vi "Example SPI ADXL345.vi"() -> ()   [LabVIEW 2021]
uses:
  <vilib>/platform/TimedLoop/XDataNode/XDataNode.xnode
  <vilib>/Platform/TimedLoop/XDataNode/nitl_modes.ctl
  <vilib>/Platform/TimedLoop/XDataNode/XDNodeRunTimeDep.lvlib
  <vilib>/Platform/TimedLoop/XDataNode/wakeup.ctl
  <vilib>/Platform/TimedLoop/XDataNode/timing_clust.ctl
  wiringPi.lvlib
  Type Defs/SPI Dev.ctl
  Type Defs/SPI Channel.ctl
  Type Defs/SPI Device.ctl
panel:
  in  "SPI Device":T1
  out "Aceleration":cluster{dbl, dbl, dbl}(graph)
  in  "stop":bool
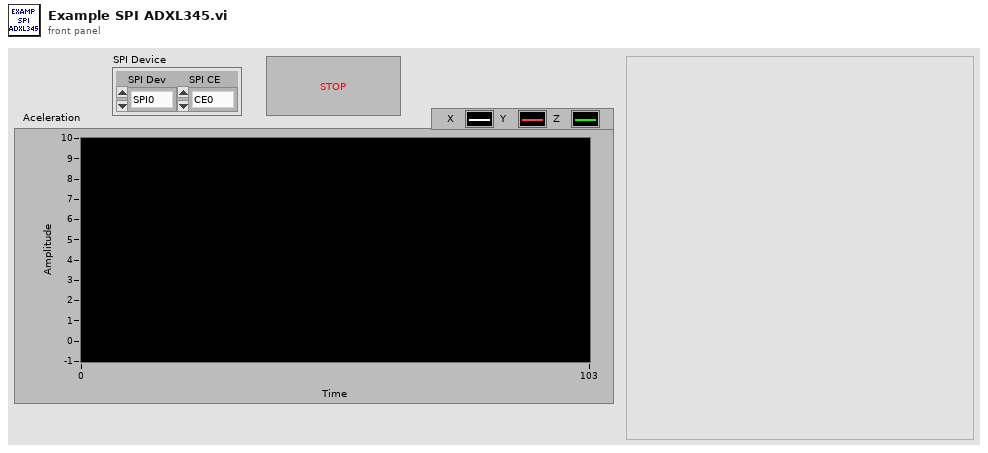
[diagram p1: front panel]
types:
  T1 = typedef "wiringPi.lvlib/SPI Device.ctl" = cluster{"SPI Dev":T2, "SPI CE":T3}
  T2 = typedef "wiringPi.lvlib/SPI Dev.ctl" = enum32{"SPI0", "SPI1"}
  T3 = typedef "wiringPi.lvlib/SPI Channel.ctl" = enum32{"CE0", "CE1", "CE2"}
  T4 = enum8{"DEVID", "-1-", "-2-", "-3-", "-4-", "-5-", "-6-", "-7-", "-8-", "-9-", "-A-", "-B-", "-C-", "-D-", "-E-", "-F-", "-10-", "-11-", "-12-", "-13-", "-14-", "-15-", "-16", "-17", "-18-", "-19-", "-1A-", "-1B-", "-1C-", "THRESH_TAP", "OFSX", "OFSY", "OFSZ", "DUR", "Latent", "Window", "THRESH_ACT", "THRESH_INACT", "TIME_INACT", "ACT_INACT_CTL", "THRESH_FF", "TIME_FF", "TAP_AXES", "ACT_TAP_STATUS", "BW_RATE", "POWER_CTL", "INT_ENABLE", "INT_MAP", "INT_SOURCE", "DATA_FORMAT", "DATAX0", "DATAX1", "DATAY0", "DATAY1", "DATAZ0", "DATAZ1", "FIFO_CTL", "FIFO_STATUS"}
  T5 = typedef "XDNodeRunTimeDep.lvlib/timing_clust.ctl" = cluster{"Expected End [f-1]":u64, "Actual End [f-1]":u64, "Finished Late? [f-1]":bool, "Expected End [i-1]":u64, "Actual End [i-1]":u64, "Finished Late? [i-1]":bool, "Expected Start [i]":u64, "Actual Start [i]":u64, "Expected Start [f]":u64, "Actual Start [f]":u64, "Source Name":string, "Structure Name":string, "Period":i64, "Deadline":i64, "Offset":i64, "Start":i64, "Priority":i32, "Timeout":i32, "Mode":T6, "Wakeup Reason":T7, "Error":errorcluster, "Source Type":string, "Secondary Source Type":string, "Global End Time":u64, "Global Start Time":u64, "Frame Duration":u64, "Iteration Duration":u64, "Assigned CPU":i32, "I/O Scan Engine Mode":u32}
  T6 = typedef "XDNodeRunTimeDep.lvlib/nitl_modes.ctl" = enum32{"No Change", "Process missed periods, maintain original phase", "Discard missed periods, maintain original phase", "Process missed periods, ignore original phase", "Discard missed periods, ignore original phase"}
  T7 = typedef "XDNodeRunTimeDep.lvlib/wakeup.ctl" = enum32{"Normal", "Aborted", "Asynchronous wakeup", "Timing source error", "Timed loop error", "Timeout"}
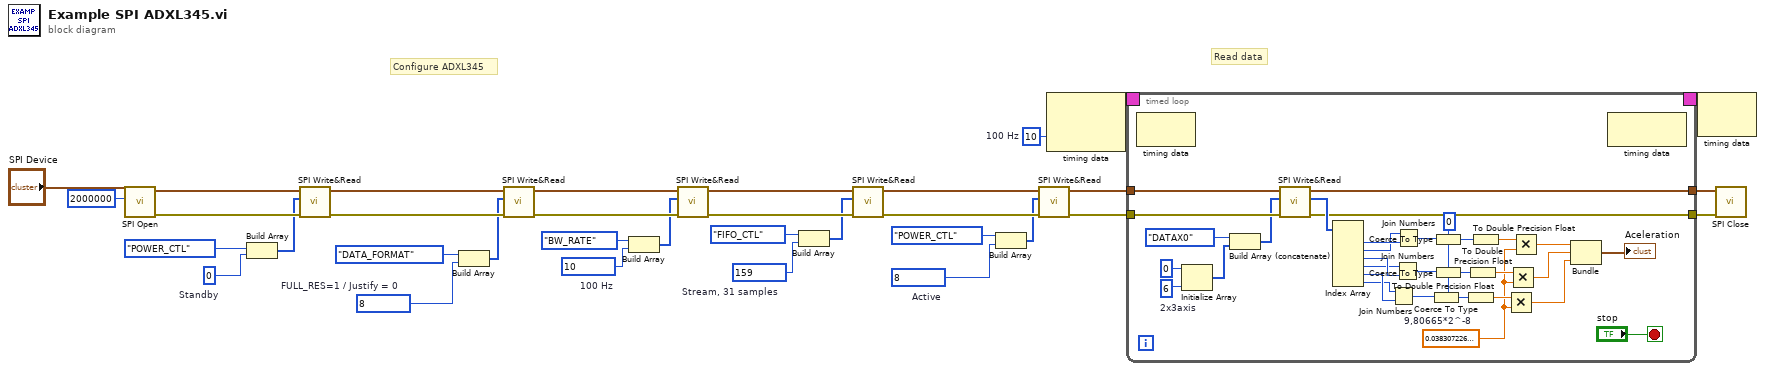
[diagram p0: block diagram]
diagram:
  w26 = i64 10  # 100 Hz
  w13 = u8 10  # 100 Hz
  w8 = u8 159  # Stream, 31 samples
  w17 = u8 8  # FULL_RES=1 / Justify = 0
  w6 = u8 8  # Active
  w21 = u8 0  # Standby
  # "Read data"
  # "Configure ADXL345"
  n1 = call "SPI Open.vi"("Speed"=2000000, "SPI Device"="SPI Device") -> ("error out"=w34:errorcluster, "SPI Device out"=w19:T1)  [unwired: 8 in]
  n2 = Build Array(T4."POWER_CTL" ("Dirección"), w21) -> (w20:u8[])
  n3 = call "SPI Write&Read.vi"("error in (no error)"=w34, "Data to Write"=w20, "SPI Device"=w19) -> ("error out"=w29:errorcluster, "SPI Device out"=w15:T1)  [unwired: 6 in, 1 out]
  n4 = Build Array(T4."DATA_FORMAT" ("Dirección"), w17) -> (w16:u8[])
  n5 = call "SPI Write&Read.vi"("error in (no error)"=w29, "Data to Write"=w16, "SPI Device"=w15) -> ("error out"=w33:errorcluster, "SPI Device out"=w14:T1)  [unwired: 6 in, 1 out]
  n6 = Build Array(T4."BW_RATE" ("Dirección"), w13) -> (w11:u8[])
  n7 = call "SPI Write&Read.vi"("error in (no error)"=w33, "Data to Write"=w11, "SPI Device"=w14) -> ("error out"=w31:errorcluster, "SPI Device out"=w3:T1)  [unwired: 6 in, 1 out]
  n8 = Build Array(T4."FIFO_CTL" ("Dirección"), w8) -> (w10:u8[])
  n9 = call "SPI Write&Read.vi"("error in (no error)"=w31, "Data to Write"=w10, "SPI Device"=w3) -> ("error out"=w32:errorcluster, "SPI Device out"=w4:T1)  [unwired: 6 in, 1 out]
  n10 = Build Array(T4."POWER_CTL" ("Dirección"), w6) -> (w5:u8[])
  n11 = call "SPI Write&Read.vi"("error in (no error)"=w32, "Data to Write"=w5, "SPI Device"=w4) -> ("error out"=w30:errorcluster, "SPI Device out"=w2:T1)  [unwired: 6 in, 1 out]
  n12 = node-c288(w26) -> (w28:T5)  [unwired: 1 in]
  n13 = timed-loop {
    timing: w28 -> [_]
    timing-out: [_] -> w27
    tunnel: w30 -> [w66]
    tunnel: [w46] -> w1
    tunnel: [w45] -> w25
    tunnel: w2 -> [w40]
    stop <- "stop" stop-if-true
    w51 = i16 0 ("number")
    w48 = 0.0383072265625  # 9,80665*2^-8
    w38 = u32 6  # 2x3axis
    n14 = node-c288() -> ()  [unwired: 1 in, 1 out]
    n15 = Initialize Array(u8 0 ("element"), w38) -> (w36:u8[])
    n16 = Build Array (concatenate)(T4."DATAX0" ("Address"), w36) -> (w35:u8[])
    n17 = call "SPI Write&Read.vi"("error in (no error)"=w66, "Data to Write"=w35, "SPI Device"=w40) -> ("error out"=w45:errorcluster, "Data readed"=w62:u8[], "SPI Device out"=w46:T1)  [unwired: 6 in]
    n18 = Index Array(array=w62) -> (element #1=w61:u8, element #2=w60:u8, element #3=w53:u8, element #4=w52:u8, element #5=w50:u8, element #6=w49:u8)  [unwired: 6 in]
    n19 = Join Numbers(hi=w49, lo=w50) -> ((hi.lo)=w55:u16)
    n20 = Join Numbers(hi=w52, lo=w53) -> ((hi.lo)=w54:u16)
    n21 = Join Numbers(hi=w60, lo=w61) -> ((hi.lo)=w63:u16)
    n22 = Coerce To Type(0:w55, 1:w51) -> (2:w56:i16)
    n23 = Coerce To Type(0:w63, 1:w51) -> (2:w64:i16)
    n24 = Coerce To Type(0:w54, 1:w51) -> (2:w59:i16)
    n25 = To Double Precision Float(number=w56) -> (double precision float=w57:dbl)
    n26 = To Double Precision Float(number=w59) -> (double precision float=w58:dbl)
    n27 = To Double Precision Float(number=w64) -> (double precision float=w65:dbl)
    n28 = Multiply(x=w57, y=w48) -> (x*y=w42:dbl)
    n29 = Multiply(x=w58, y=w48) -> (x*y=w43:dbl)
    n30 = Multiply(x=w65, y=w48) -> (x*y=w44:dbl)
    n31 = Bundle(w44, w43, w42) -> (→"Aceleration":cluster{dbl, dbl, dbl})  [unwired: 1 in]
    n32 = node-c288() -> ()  [unwired: 1 in, 1 out]
  }
  n33 = node-c288(w27) -> ()  [unwired: 1 out]
  n34 = call "SPI Close.vi"("error in (no error)"=w25, "SPI Device"=w1) -> ()  [unwired: 9 in, 1 out]
